vi "Update Serial Input.vi"(7 "Serial Input Ref":refnum<vi>, 8 "error in (no error)":errorcluster, 11 "SERIAL INPUT (SI) Ref":refnum<vi>) -> (0 "error out":errorcluster)   [LabVIEW 2025, in "I2C Bus Monitor UI.lvlib"]
uses:
  I2C Bus Monitor UI.lvlib
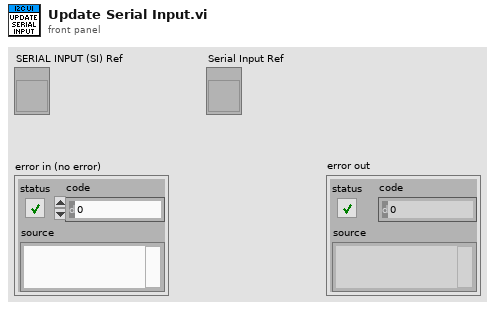
[diagram p1: front panel]
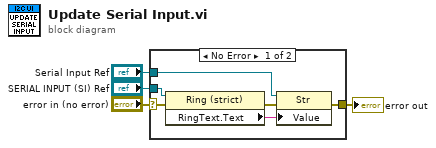
[diagram p0: block diagram]
diagram:
  n1 = case shown="No Error" "error in (no error)" {
    selector: "error in (no error)" -> [w7 w11]
    tunnel: "Serial Input Ref" -> [w9 _]
    tunnel: "SERIAL INPUT (SI) Ref" -> [w6 _]
    tunnel: [w5 w11] -> w1
    frame No Error {
      n2 = property class="Ring (strict)"(reference=w6, error in=w7) -> (error out=w8:errorcluster, "RingText.Text"=w10:string)  [unwired: 1 out]
      n3 = property class="Str"(reference=w9, error in=w8, "Value"=w10) -> (error out=w5:errorcluster)  [unwired: 1 out]
    }
    frame Error {
    }
  }
  "error out" <- w1
